vi "ExportResults.vi"(8 "error in (no error)":errorcluster, 11 "CDependencyInspector in":refnum<class "CDependencyInspection.lvclass">) -> (0 "error out":errorcluster, 3 "CDependencyInspector out":refnum<class "CDependencyInspection.lvclass">)   [LabVIEW 2020, in "DependencyInspection.lvlib" / "CDependencyInspection.lvclass"]
uses:
  CDependencyInspection.lvclass
  ExtensionInterfaces/IExporter/ExportType.ctl
  CDependencyInspection.lvclass/CDependencyInspection.ctl
  ErrorManager/ErrorManager/ErrorType.ctl
  ExtensionInterfaces/IExporter/IExporter.lvclass
  CReporter/CReporter.lvclass
  CDependencyList/CDependencyList.lvclass
  CRuleList/CRuleList.lvclass
  ErrorManager/ErrorManager/ErrorManager.lvclass
  LabVIEWObjectInterfaces/IErrorManager/IErrorManager.lvclass
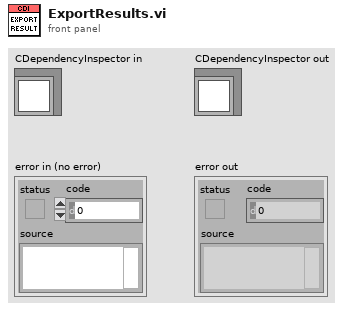
[diagram p1: front panel]
types:
  T1 = typedef "ExtensionInterfaces.lvlib/IExporter.lvclass/ExportType.ctl" = enum16{"Dependencies", "Rules", "Invalid dependencies", "Concessions", "Undeclared"}
  T2 = typedef "LabVIEWObjectInterfaces.lvlib/IErrorManager.lvclass/ErrorType.ctl" = enum16{"Info", "Warning", "Error"}
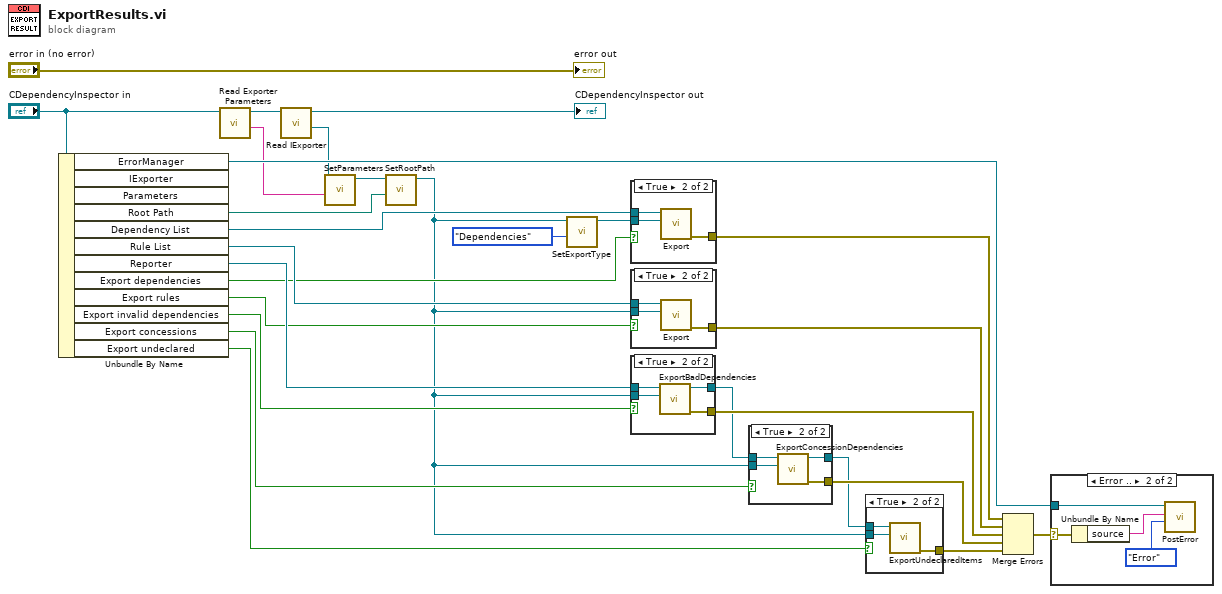
[diagram p0: block diagram]
diagram:
  n1 = Unbundle By Name("CDependencyInspector in") -> ("ErrorManager"=w23:refnum<class "ErrorManager.lvclass">, "Root Path"=w10:path, "Dependency List"=w11:refnum<class "CDependencyList.lvclass">, "Rule List"=w28:refnum<class "CRuleList.lvclass">, "Reporter"=w19:refnum<class "CReporter.lvclass">, "Export dependencies"=w16:bool, "Export rules"=w15:bool, "Export invalid dependencies"=w14:bool, "Export concessions"=w13:bool, "Export undeclared"=w12:bool)  [unwired: 2 out]
  n2 = call-dynamic "Read Exporter Parameters.vi"("CDependencyInspection in"="CDependencyInspector in") -> ("Parameters"=w4:string, "CDependencyInspection out"=w3:refnum<class "CDependencyInspection.lvclass">)  [unwired: 9 in]
  n3 = call-dynamic "Read IExporter.vi"("CDependencyInspection in"=w3) -> ("IExporter"=w1:refnum<class "IExporter.lvclass">, "CDependencyInspection out"=→"CDependencyInspector out":refnum<class "CDependencyInspection.lvclass">)  [unwired: 9 in]
  n4 = call-dynamic "SetParameters.vi"("Parameters"=w4, "IExporter in"=w1) -> ("IExporter out"=w9:refnum<class "IExporter.lvclass">)  [unwired: 8 in, 1 out]
  n5 = call-dynamic "SetRootPath.vi"("Root path"=w10, "IExporter in"=w9) -> ("IExporter out"=w8:refnum<class "IExporter.lvclass">)  [unwired: 8 in, 1 out]
  n6 = call-dynamic "SetExportType.vi"("Export type"=ExportType."Dependencies", "IExporter in"=w8) -> ("IExporter out"=w7:refnum<class "IExporter.lvclass">)  [unwired: 8 in, 1 out]
  n7 = case shown="True" w16 {
    tunnel: w11 -> [_ w31]
    tunnel: [_ w30] -> w25
    tunnel: w7 -> [_ w29]
    frame False {
    }
    frame True {
      n8 = call-dynamic "Export.vi"("IExporter"=w29, "CDependencyList in"=w31) -> ("error out"=w30:errorcluster)  [unwired: 8 in, 1 out]
    }
  }
  n9 = case shown="True" w15 {
    tunnel: w28 -> [_ w34]
    tunnel: [_ w33] -> w26
    tunnel: w8 -> [_ w32]
    frame False {
    }
    frame True {
      n10 = call-dynamic "Export.vi"("IExporter"=w32, "CRuleList in"=w34) -> ("error out"=w33:errorcluster)  [unwired: 8 in, 1 out]
    }
  }
  n11 = case shown="True" w14 {
    tunnel: [_ w39] -> w22
    tunnel: w19 -> [w35 w38]
    tunnel: [w35 w37] -> w18
    tunnel: w8 -> [_ w36]
    frame False {
    }
    frame True {
      n12 = call-dynamic "ExportBadDependencies.vi"("IExporter"=w36, "CReporter in"=w38) -> ("error out"=w39:errorcluster, "CReporter out"=w37:refnum<class "CReporter.lvclass">)  [unwired: 8 in]
    }
  }
  n13 = case shown="True" w13 {
    tunnel: [_ w44] -> w20
    tunnel: w18 -> [w40 w43]
    tunnel: [w40 w42] -> w17
    tunnel: w8 -> [_ w41]
    frame False {
    }
    frame True {
      n14 = call-dynamic "ExportConcessionDependencies.vi"("IExporter"=w41, "CReporter in"=w43) -> ("error out"=w44:errorcluster, "CReporter out"=w42:refnum<class "CReporter.lvclass">)  [unwired: 8 in]
    }
  }
  n15 = case shown="True" w12 {
    tunnel: [_ w47] -> w21
    tunnel: w17 -> [_ w46]
    tunnel: w8 -> [_ w45]
    frame False {
    }
    frame True {
      n16 = call-dynamic "ExportUndeclaredItems.vi"("IExporter"=w45, "CReporter in"=w46) -> ("error out"=w47:errorcluster)  [unwired: 8 in, 1 out]
    }
  }
  n17 = Merge Errors(w25, w26, w22, w20, w21) -> (w24:errorcluster)
  n18 = case shown="Error .." w24 {
    selector: w24 -> [_ w50]
    tunnel: w23 -> [_ w51]
    frame No Error {
    }
    frame Error {
      n19 = Unbundle By Name(w50) -> ("source"=w49:string)
      n20 = call-dynamic "PostError.vi"("Type"=ErrorType."Error", "Message"=w49, "ErrorManager in"=w51) -> ()  [unwired: 7 in, 2 out]
    }
  }
  "error out" <- "error in (no error)"
